vi "FSK Demodulator.vi"(0 "FSK Modulated Signal":dbl[](array[numeric]), 1 "Sampling Frequency (Fs)":dbl, 2 "Lower Frequency (f0)":dbl, 3 "Higher Frequency (f1)":dbl, 4 "Samples per Bit":i32) -> (5 "Recovered Binary Signal":dbl[](array[numeric]))   [LabVIEW 2026]
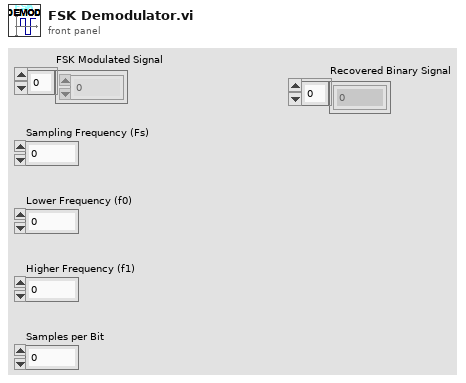
[diagram p1: front panel]
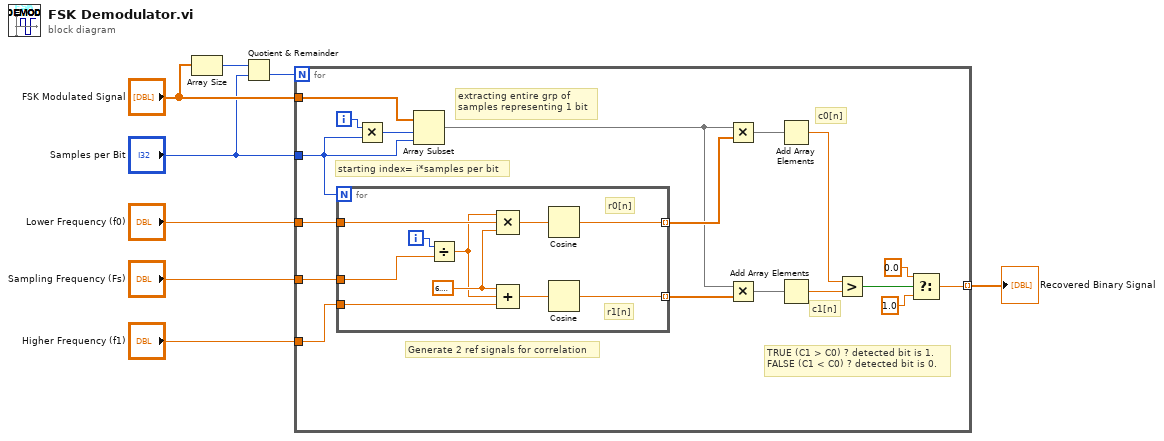
[diagram p0: block diagram]
diagram:
  n1 = Array Size(array="FSK Modulated Signal") -> (size(s)=w8:i32)
  n2 = Quotient & Remainder(x=w8, y="Samples per Bit") -> (floor(x/y)=w7:i32)  [unwired: 1 out]
  n3 = for {
    N: w7 -> [_]
    tunnel: "Samples per Bit" -> [w23]
    tunnel: "FSK Modulated Signal" -> [w25]
    tunnel: "Sampling Frequency (Fs)" -> [w22]
    tunnel: "Lower Frequency (f0)" -> [w21]
    tunnel: "Higher Frequency (f1)" -> [w20]
    tunnel: [w9] -> w2 mode=indexing
    i -> [w26]
    # "starting index= i*samples per bit"
    # "extracting entire grp of \nsamples representing 1 bit"
    # "TRUE (C1 > C0) ? detected bit is 1.\nFALSE (C1 < C0) ? detected bit is 0."
    # "c1[n]"
    # "c0[n]"
    # "Generate 2 ref signals for correlation"
    n4 = for {
      N: w23 -> [_]
      tunnel: w22 -> [w35]
      tunnel: w21 -> [w34]
      tunnel: [w32] -> w19 mode=indexing
      tunnel: w20 -> [w29]
      tunnel: [w27] -> w17 mode=indexing
      i -> [w36]
      w31 = 6.283185307179586
      # "r1[n]"
      # "r0[n]"
      n5 = Divide(x=w36, y=w35) -> (x/y=w30:dbl)
      n6 = Compound Arithmetic op=MULTIPLY(w30, w34, w31) -> (w33:dbl)
      n7 = Compound Arithmetic op=ADD(w31, w30, w29) -> (w28:dbl)
      n8 = Cosine(x=w33) -> (cos(x)=w32:dbl)
      n9 = Cosine(x=w28) -> (cos(x)=w27:dbl)
    }
    n10 = Multiply(x=w26, y=w23) -> (x*y=w24:i32)
    n11 = Array Subset(array=w25, index=w24, length=w23) -> (w16:dbl[])
    n12 = Multiply(x=w16, y=w19) -> (x*y=w18:dbl[])
    n13 = Multiply(x=w16, y=w17) -> (x*y=w15:dbl[])
    n14 = Add Array Elements(numeric array=w18) -> (sum=w14:dbl)
    n15 = Add Array Elements(numeric array=w15) -> (sum=w13:dbl)
    n16 = Greater?(x=w14, y=w13) -> (0:w12:bool)
    n17 = Select(t=0.0, s=w12, f=1.0) -> (s? t:f=w9:dbl)
  }
  "Recovered Binary Signal" <- w2
